vi "Set LEDs.vi"(8 "error in (no error)":errorcluster, 10 "LED Array":u32[][](array[colorbox]), 11 "LINX-SenseHat in":refnum<class "LINX-SenseHat.lvclass">) -> (0 "error out":errorcluster, 3 "LINX-SenseHat out":refnum<class "LINX-SenseHat.lvclass">)   [LabVIEW 2020, in "LINX-SenseHat.lvclass"]
doc: "Sets the 8x8 LED matrix on the Sense Hat. Required the kernel framebuffer driver for the sense-hat to be disabled to function."
uses:
  LINX-SenseHat.lvclass
  LINX-SenseHat.lvclass/LINX-SenseHat.ctl
  LINX I2C/LINX I2C.lvclass
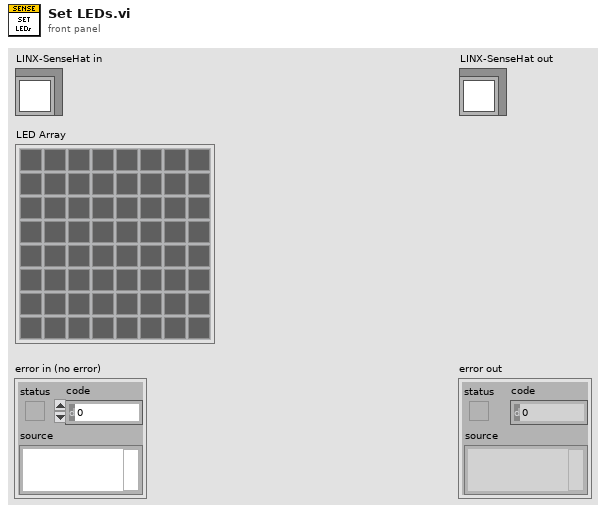
[diagram p1: front panel]
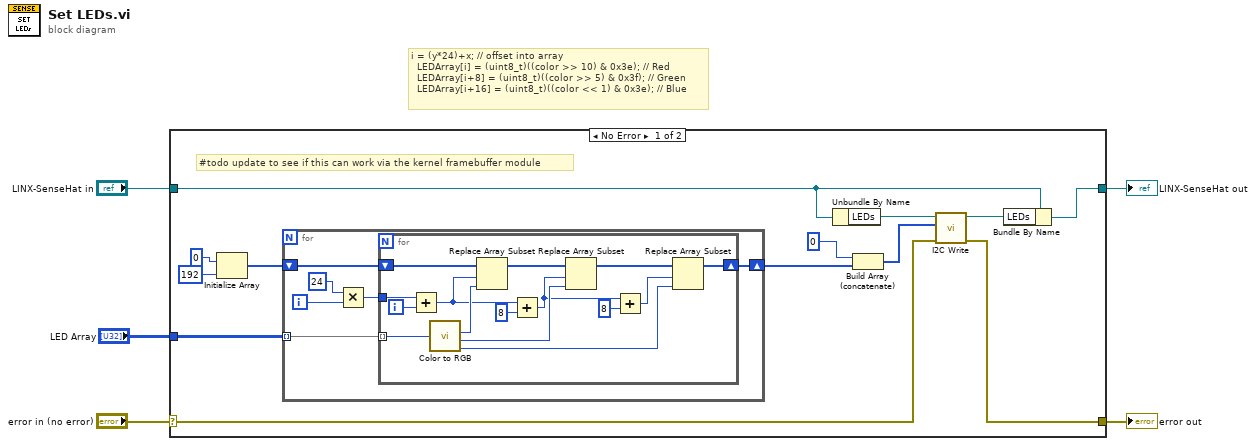
[diagram p0: block diagram]
diagram:
  # "i = (y*24)+x; // offset into array\n\t\tLEDArray[i] = (uint8_t)((color >> 10) & 0x3e); // Red\n\t\tLEDArray[i+8] = (uint8_t)((color >> 5) & 0x3f); // Green\n\t\tLEDArray[i+16] = (uint8_t)((color << 1) & 0x3e); // Blue"
  n1 = case shown="No Error" "error in (no error)" {
    selector: "error in (no error)" -> [w14 w41]
    tunnel: [w13 w41] -> w4
    tunnel: [w15 w40] -> w2
    tunnel: "LINX-SenseHat in" -> [w16 w40]
    tunnel: "LED Array" -> [w11 _]
    frame No Error {
      # "#todo update to see if this can work via the kernel framebuffer module"
      n2 = Initialize Array(u8 0, 192) -> (w7:u8[])
      n3 = for {
        tunnel: w11 -> [w24] mode=indexing
        shift-right: [w22] -> w6
        shift-left: w7 -> [w23]
        i -> [w21]
        n4 = Multiply(x=24, y=w21) -> (x*y=w19:i32)
        n5 = for {
          tunnel: w24 -> [w39] mode=indexing
          shift-right: [w35] -> w22
          shift-left: w23 -> [w38]
          tunnel: w19 -> [w37]
          i -> [w33]
          n6 = Add(x=w37, y=w33) -> (x+y=w29:i32)
          n7 = call <vilib>:"Color to RGB.vi"("Color"=w39) -> ("R"=w32:u8, "G"=w31:u8, "B"=w30:u8)  [unwired: 1 out]
          n8 = Replace Array Subset(array=w38, new element=w32, index=w29) -> (w36:u8[])
          n9 = Add(x=w29, y=8) -> (x+y=w26:i32)
          n10 = Replace Array Subset(array=w36, new element=w31, index=w26) -> (w34:u8[])
          n11 = Add(x=w26, y=8) -> (x+y=w25:i32)
          n12 = Replace Array Subset(array=w34, new element=w30, index=w25) -> (w35:u8[])
        }
      }
      n13 = Unbundle By Name(w16) -> ("LEDs"=w18:refnum<class "LINX I2C.lvclass">)
      n14 = Build Array (concatenate)(u8 0, w6) -> (w12:u8[])
      n15 = call "I2C Write.vi"("error in (no error)"=w14, "Bytes to Write"=w12, "LINX I2C in"=w18) -> ("error out"=w13:errorcluster, "LINX I2C out"=w17:refnum<class "LINX I2C.lvclass">)  [unwired: 7 in]
      n16 = Bundle By Name(cluster=w16, "LEDs"=w17) -> (w15:refnum<class "LINX-SenseHat.lvclass">)
    }
    frame Error {
    }
  }
  "error out" <- w4
  "LINX-SenseHat out" <- w2
